vi "DataTransHD220(SubVI).vi"(8 "error in (no error)":errorcluster caption="에러 입력(에러 없음)", 11 "배열 4":u16[][](array[numeric])) -> (0 "error out":errorcluster caption="에러 출력", 3 "배열":sgl[](array[numeric]))   [LabVIEW 2019]
panel:
  out "출력 배열":sgl[](array[numeric])
  in  "배열 3":sgl[](array[numeric])
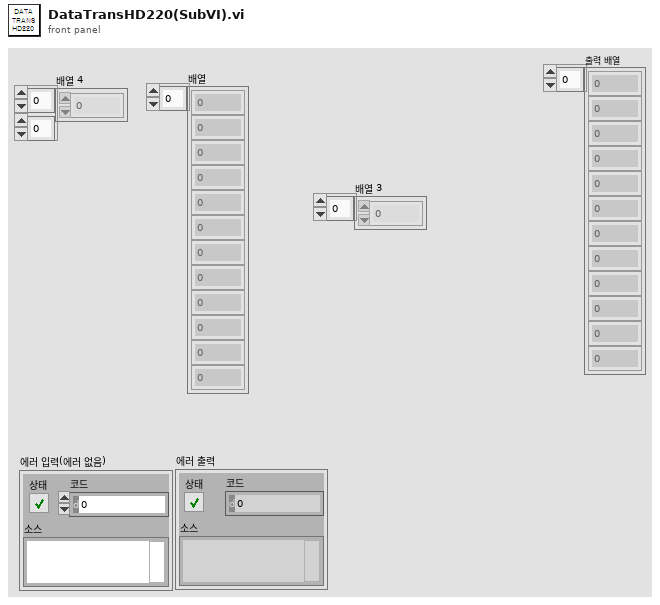
[diagram p1: front panel]
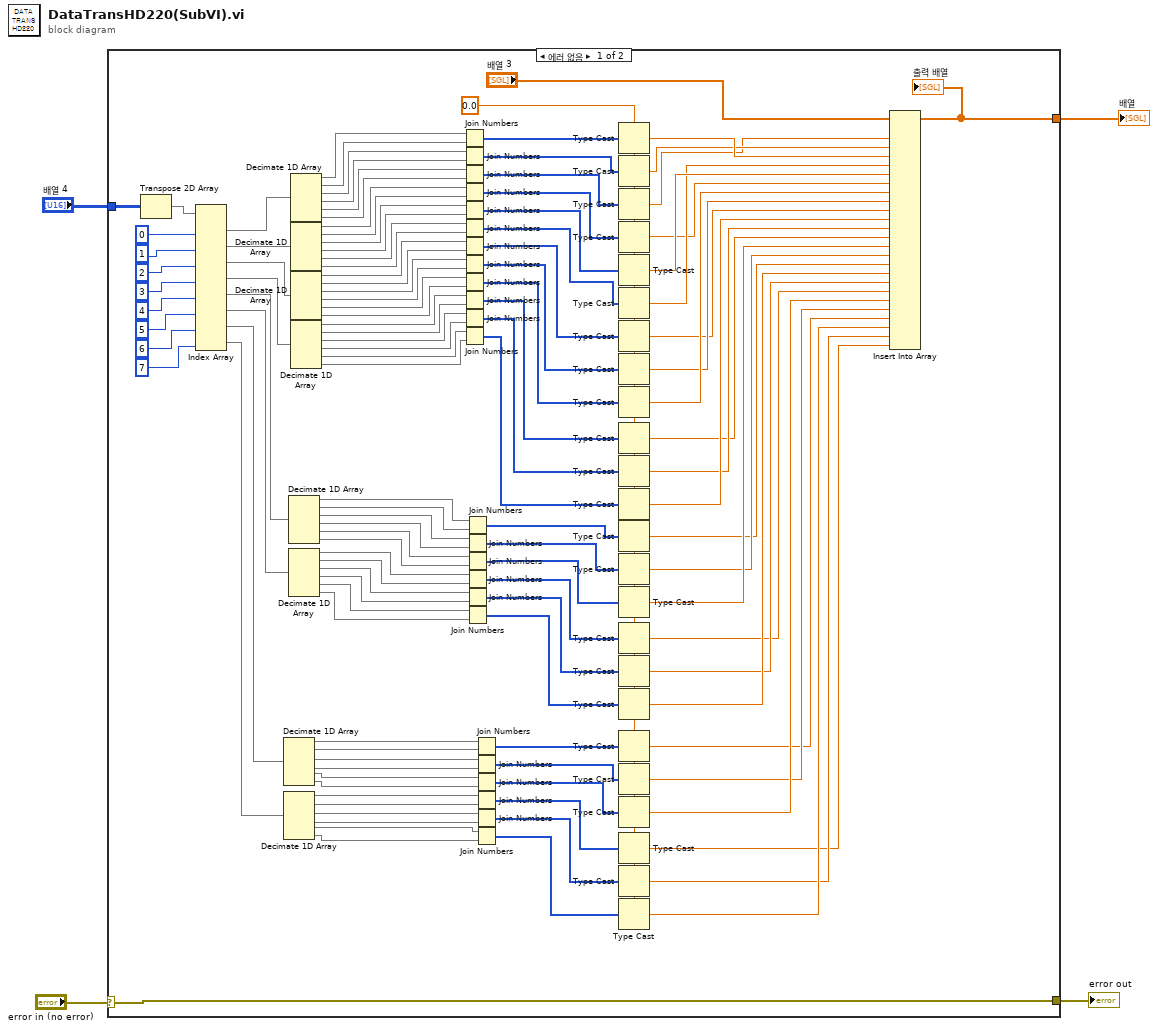
[diagram p0: block diagram]
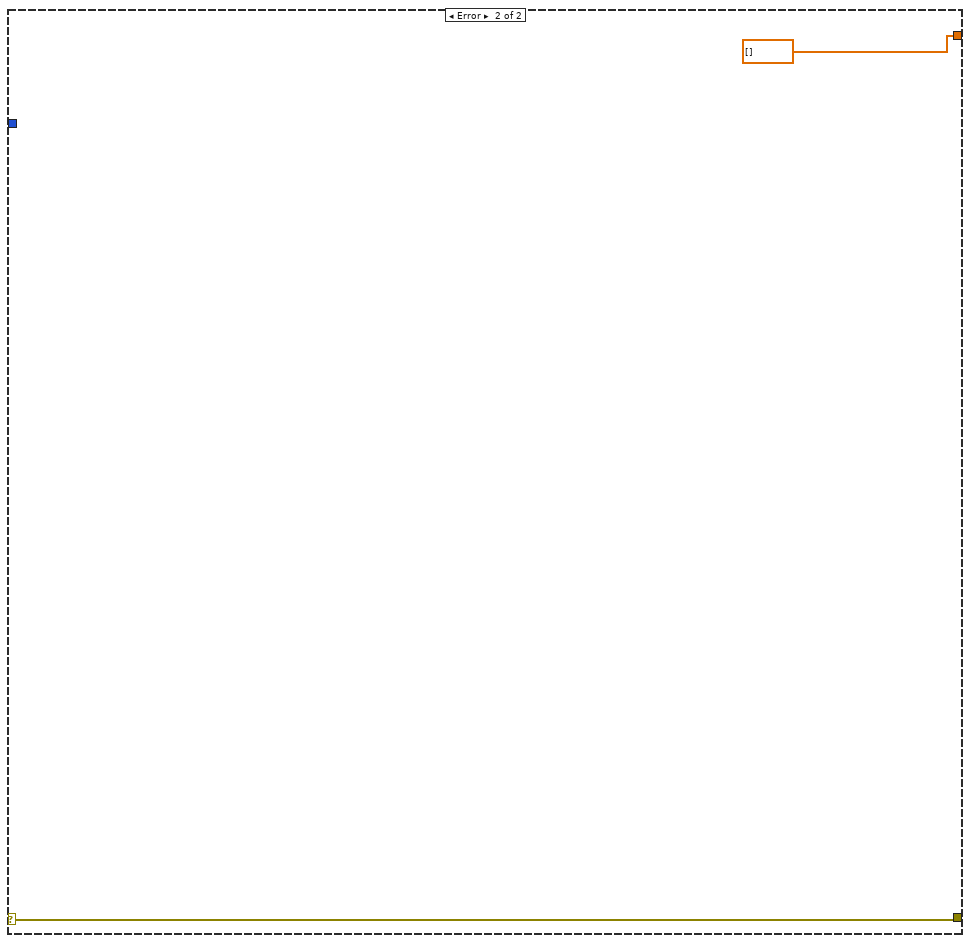
[diagram p2: hidden frame]
diagram:
  n1 = case shown="에러 없음" "error in (no error)" {
    selector: "error in (no error)" -> [w122 w124]
    tunnel: [w122 w124] -> w3
    tunnel: "배열 4" -> [w114 _]
    tunnel: [w74 sgl[] [] ("배열 3")] -> w1
    frame No Error {
      w17 = sgl 0.0
      n2 = Transpose 2D Array(2D array=w114) -> (transposed array=w121:u16[][])
      n3 = Index Array(array=w121, index (col) #1=0 ("비활성화된 인덱스 (열)"), index (col) #2=1 ("인덱스 (열)"), index (col) #3=2 ("인덱스 (열)"), index (col) #4=3 ("인덱스 (열)"), index (col) #5=4 ("인덱스 (열)"), index (col) #6=5 ("인덱스 (열)"), index (col) #7=6 ("인덱스 (열)"), index (col) #8=7 ("인덱스 (열)")) -> (element #1=w116:u16[], element #2=w107:u16[], element #3=w106:u16[], element #4=w105:u16[], element #5=w59:u16[], element #6=w58:u16[], element #7=w31:u16[], element #8=w30:u16[])  [unwired: 8 in]
      n4 = Decimate 1D Array(w31) -> (w29:u16[], w28:u16[], w27:u16[], w26:u16[], w25:u16[], w24:u16[])
      n5 = Decimate 1D Array(w30) -> (w23:u16[], w22:u16[], w21:u16[], w20:u16[], w19:u16[], w18:u16[])
      n6 = Decimate 1D Array(w59) -> (w57:u16[], w56:u16[], w55:u16[], w54:u16[], w53:u16[], w52:u16[])
      n7 = Decimate 1D Array(w58) -> (w51:u16[], w50:u16[], w49:u16[], w48:u16[], w47:u16[], w46:u16[])
      n8 = Decimate 1D Array(w116) -> (w113:u16[], w112:u16[], w111:u16[], w110:u16[], w109:u16[], w108:u16[])
      n9 = Decimate 1D Array(w107) -> (w104:u16[], w103:u16[], w102:u16[], w101:u16[], w100:u16[], w99:u16[])
      n10 = Decimate 1D Array(w106) -> (w98:u16[], w97:u16[], w96:u16[], w95:u16[], w94:u16[], w93:u16[])
      n11 = Decimate 1D Array(w105) -> (w92:u16[], w91:u16[], w90:u16[], w89:u16[], w88:u16[], w87:u16[])
      n12 = Join Numbers(hi=w113, lo=w112) -> ((hi.lo)=w119:u32[])
      n13 = Join Numbers(hi=w111, lo=w110) -> ((hi.lo)=w117:u32[])
      n14 = Join Numbers(hi=w109, lo=w108) -> ((hi.lo)=w115:u32[])
      n15 = Join Numbers(hi=w104, lo=w103) -> ((hi.lo)=w86:u32[])
      n16 = Join Numbers(hi=w102, lo=w101) -> ((hi.lo)=w85:u32[])
      n17 = Join Numbers(hi=w100, lo=w99) -> ((hi.lo)=w84:u32[])
      n18 = Join Numbers(hi=w98, lo=w97) -> ((hi.lo)=w83:u32[])
      n19 = Join Numbers(hi=w96, lo=w95) -> ((hi.lo)=w82:u32[])
      n20 = Join Numbers(hi=w94, lo=w93) -> ((hi.lo)=w81:u32[])
      n21 = Join Numbers(hi=w92, lo=w91) -> ((hi.lo)=w80:u32[])
      n22 = Join Numbers(hi=w90, lo=w89) -> ((hi.lo)=w79:u32[])
      n23 = Join Numbers(hi=w88, lo=w87) -> ((hi.lo)=w78:u32[])
      n24 = Join Numbers(hi=w57, lo=w56) -> ((hi.lo)=w45:u32[])
      n25 = Join Numbers(hi=w55, lo=w54) -> ((hi.lo)=w44:u32[])
      n26 = Join Numbers(hi=w53, lo=w52) -> ((hi.lo)=w43:u32[])
      n27 = Join Numbers(hi=w51, lo=w50) -> ((hi.lo)=w42:u32[])
      n28 = Join Numbers(hi=w49, lo=w48) -> ((hi.lo)=w41:u32[])
      n29 = Join Numbers(hi=w47, lo=w46) -> ((hi.lo)=w40:u32[])
      n30 = Join Numbers(hi=w29, lo=w28) -> ((hi.lo)=w16:u32[])
      n31 = Join Numbers(hi=w27, lo=w26) -> ((hi.lo)=w15:u32[])
      n32 = Join Numbers(hi=w25, lo=w24) -> ((hi.lo)=w14:u32[])
      n33 = Join Numbers(hi=w23, lo=w22) -> ((hi.lo)=w13:u32[])
      n34 = Join Numbers(hi=w21, lo=w20) -> ((hi.lo)=w12:u32[])
      n35 = Join Numbers(hi=w19, lo=w18) -> ((hi.lo)=w11:u32[])
      n36 = Type Cast(type=w17, x=w119) -> (*(type *) &x=w73:sgl)
      n37 = Type Cast(type=w17, x=w117) -> (*(type *) &x=w72:sgl)
      n38 = Type Cast(type=w17, x=w115) -> (*(type *) &x=w68:sgl)
      n39 = Type Cast(type=w17, x=w86) -> (*(type *) &x=w69:sgl)
      n40 = Type Cast(type=w17, x=w85) -> (*(type *) &x=w71:sgl)
      n41 = Type Cast(type=w17, x=w84) -> (*(type *) &x=w70:sgl)
      n42 = Type Cast(type=w17, x=w83) -> (*(type *) &x=w65:sgl)
      n43 = Type Cast(type=w17, x=w82) -> (*(type *) &x=w66:sgl)
      n44 = Type Cast(type=w17, x=w81) -> (*(type *) &x=w67:sgl)
      n45 = Type Cast(type=w17, x=w80) -> (*(type *) &x=w62:sgl)
      n46 = Type Cast(type=w17, x=w79) -> (*(type *) &x=w63:sgl)
      n47 = Type Cast(type=w17, x=w78) -> (*(type *) &x=w64:sgl)
      n48 = Type Cast(type=w17, x=w45) -> (*(type *) &x=w37:sgl)
      n49 = Type Cast(type=w17, x=w44) -> (*(type *) &x=w38:sgl)
      n50 = Type Cast(type=w17, x=w43) -> (*(type *) &x=w39:sgl)
      n51 = Type Cast(type=w17, x=w42) -> (*(type *) &x=w34:sgl)
      n52 = Type Cast(type=w17, x=w41) -> (*(type *) &x=w35:sgl)
      n53 = Type Cast(type=w17, x=w40) -> (*(type *) &x=w36:sgl)
      n54 = Type Cast(type=w17, x=w16) -> (*(type *) &x=w8:sgl)
      n55 = Type Cast(type=w17, x=w15) -> (*(type *) &x=w9:sgl)
      n56 = Type Cast(type=w17, x=w14) -> (*(type *) &x=w10:sgl)
      n57 = Type Cast(type=w17, x=w13) -> (*(type *) &x=w5:sgl)
      n58 = Type Cast(type=w17, x=w12) -> (*(type *) &x=w6:sgl)
      n59 = Type Cast(type=w17, x=w11) -> (*(type *) &x=w7:sgl)
      n60 = Insert Into Array(array="배열 3", new element #1=w68, new element #2=w72, new element #3=w73, new element #4=w70, new element #5=w71, new element #6=w69, new element #7=w67, new element #8=w66, new element #9=w65, new element #10=w64, new element #11=w63, new element #12=w62, new element #13=w39, new element #14=w38, new element #15=w37, new element #16=w36, new element #17=w35, new element #18=w34, new element #19=w10, new element #20=w9, new element #21=w8, new element #22=w7, new element #23=w6, new element #24=w5) -> (w74:sgl[])  [unwired: 1 in]
      "출력 배열" <- w74
    }
    frame Error {
    }
  }
  "error out" <- w3
  "배열" <- w1
